vi "set Gate Delay.vi"(8 "error in (no error)":errorcluster, 10 "Gate Delay Time (sec)":dbl, 11 "Keysight 9020A in":refnum<class "Keysight 9020A.lvclass">) -> (0 "error out":errorcluster, 3 "Keysight 9020A out":refnum<class "Keysight 9020A.lvclass">)   [LabVIEW 2023, in "Spectrum Analyzer.lvlib" / "Keysight 9020A.lvclass"]
uses:
  Keysight 9020A.lvclass
  Keysight 9020A.lvclass/Keysight 9020A.ctl
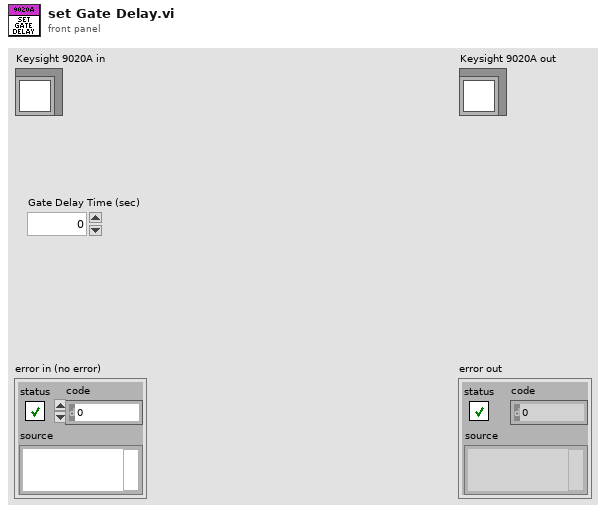
[diagram p1: front panel]
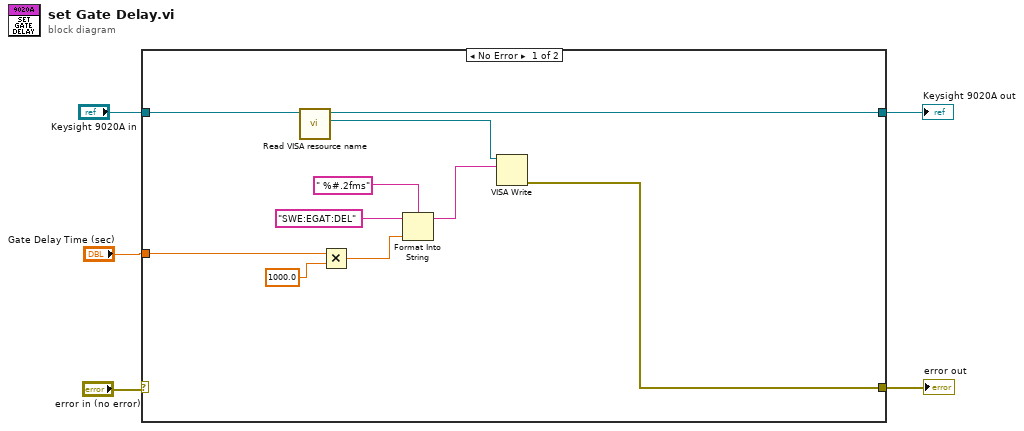
[diagram p0: block diagram]
diagram:
  n1 = case shown="No Error" "error in (no error)" {
    selector: "error in (no error)" -> [_ w16]
    tunnel: "Keysight 9020A in" -> [w8 w17]
    tunnel: [w15 w17] -> w4
    tunnel: [w7 w16] -> w2
    tunnel: "Gate Delay Time (sec)" -> [w13 _]
    frame No Error {
      n2 = call "Read VISA resource name.vi"("Keysight 9020A in"=w8) -> ("VISA resource name"=w9:refnum<visa-resource-name>, "Keysight 9020A out"=w15:refnum<class "Keysight 9020A.lvclass">)  [unwired: 8 in, 1 out]
      n3 = Multiply(x=w13, y=1000.0) -> (x*y=w11:dbl)
      n4 = Format Into String(format string=" %#.2fms", initial string="SWE:EGAT:DEL" ("string"), w11) -> (resulting string=w14:string)  [unwired: 1 in, 1 out]
      n5 = VISA Write(VISA resource name=w9, write buffer=w14) -> (error out=w7:errorcluster)  [unwired: 1 in, 2 out]
    }
    frame Error {
    }
  }
  "error out" <- w2
  "Keysight 9020A out" <- w4
